vi "hanwnag_toeplitz 3.vi"(4 "error in (no error)":errorcluster, 6 "column":cdb[](array[numeric]), 7 "row":cdb[](array[numeric])) -> (0 "error out":errorcluster, 3 "Toeplitz Array":cdb[][](array[numeric]))   [LabVIEW 2022 SP3]
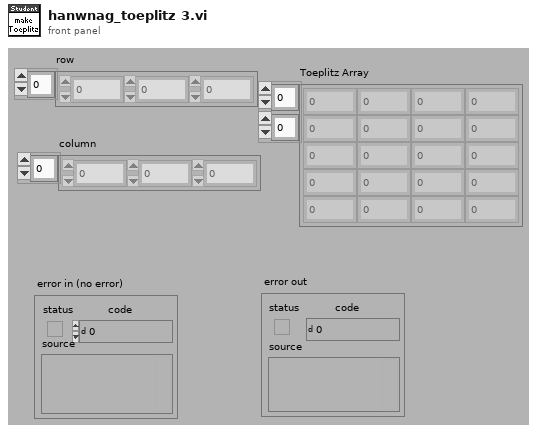
[diagram p1: front panel]
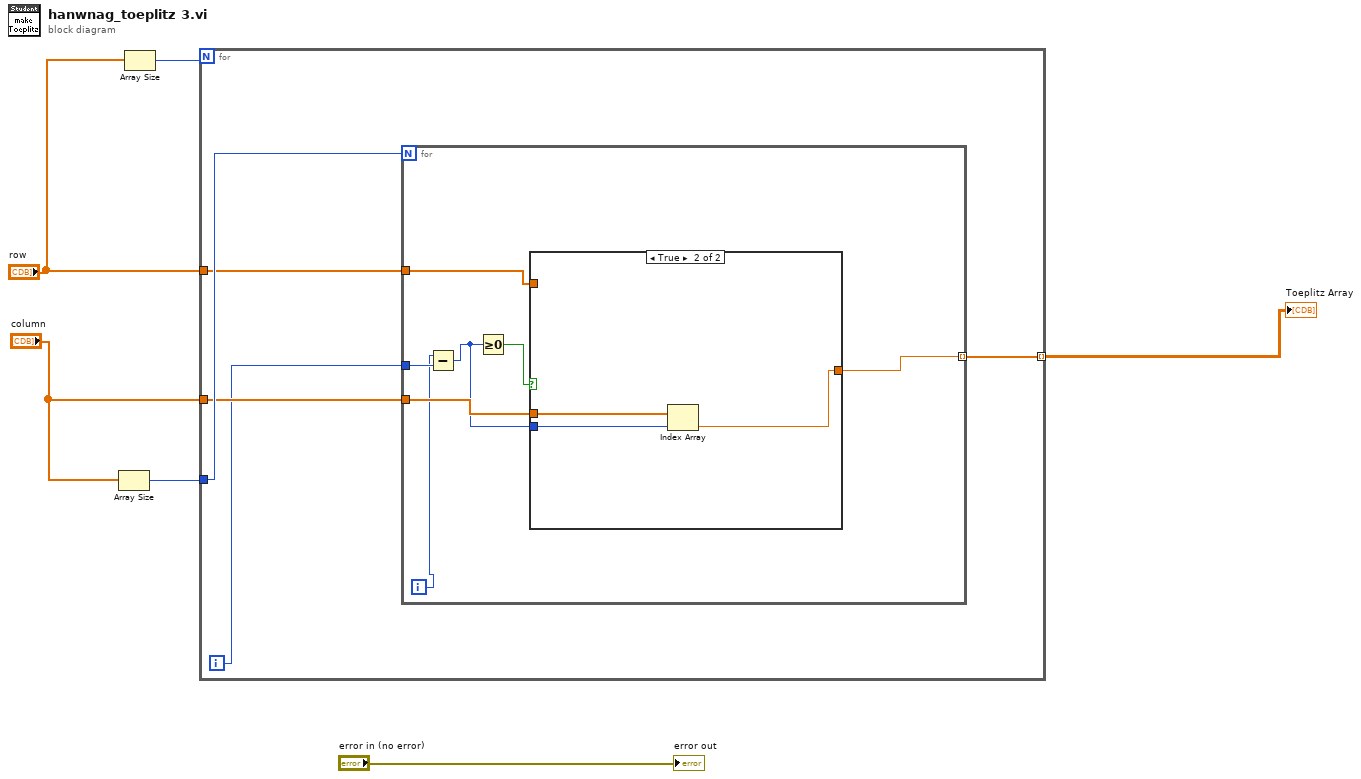
[diagram p0: block diagram]
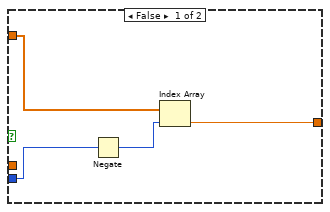
[diagram p2: hidden frame]
diagram:
  n1 = Array Size(array="column") -> (size(s)=w4:i32)
  n2 = Array Size(array="row") -> (size(s)=w6:i32)
  n3 = for {
    N: w6 -> [_]
    tunnel: w4 -> [w11]
    tunnel: "column" -> [w10]
    tunnel: "row" -> [w9]
    tunnel: [w7] -> w1 mode=indexing
    i -> [w8]
    n4 = for {
      N: w11 -> [_]
      tunnel: w10 -> [w18]
      tunnel: w9 -> [w17]
      tunnel: w8 -> [w15]
      tunnel: [w12] -> w7 mode=indexing
      i -> [w14]
      n5 = Subtract(x=w14, y=w15) -> (x-y=w13:i32)
      n6 = Greater Or Equal To 0?(x=w13) -> (x >= 0?=w16:bool)
      n7 = case shown="True" w16 {
        tunnel: w18 -> [_ w25]
        tunnel: w17 -> [w20 _]
        tunnel: w13 -> [w22 w24]
        tunnel: [w19 w23] -> w12
        frame False {
          n8 = Negate(x=w22) -> (-x=w21:i32)
          n9 = Index Array(array=w20, index=w21) -> (element=w19:cdb)
        }
        frame True {
          n10 = Index Array(array=w25, index=w24) -> (element=w23:cdb)
        }
      }
    }
  }
  "Toeplitz Array" <- w1
  "error out" <- "error in (no error)"
